vi "GOOP_AddCtrlToVIIfNeeded.vi"(11 "Ctrl VI in":refnum<vi>) -> (2 "error out":errorcluster, 3 "VI out":refnum<vi>, 5 "CtrlOut":refnum<vi>)   [LabVIEW 2020]
uses:
  <vilib>/Utility/miscctls.llb/LVPointTypeDef.ctl
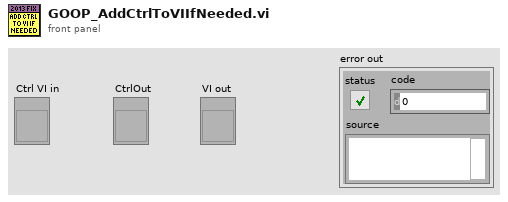
[diagram p1: front panel]
types:
  T1 = typedef "LVPointTypeDef.ctl" = cluster{"Horizontal":i16, "Vertical":i16}
  T2 = enum32{"invalid VI type", "Standard VI", "Control VI", "Global VI", "Polymorphic VI", "Configuration VI", "SubSystem", "Facade VI", "Method VI", "Statechart Diagram VI"}
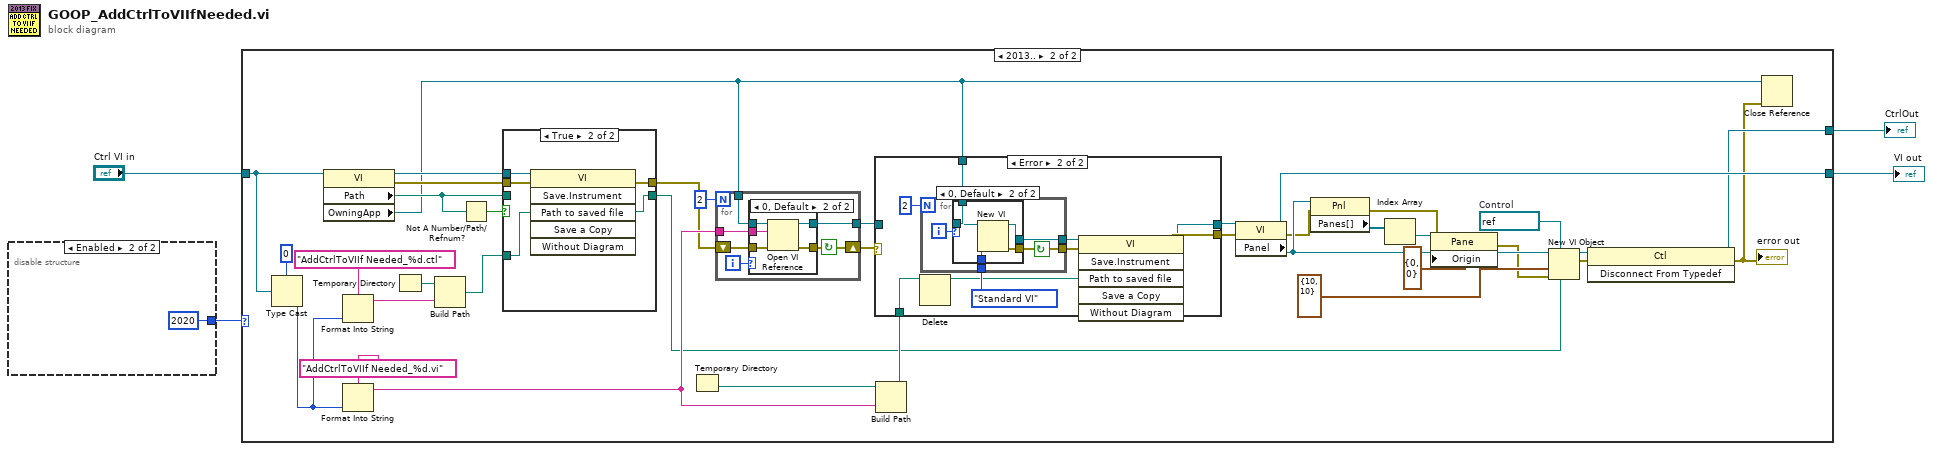
[diagram p0: block diagram]
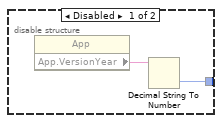
[diagram p2: hidden frame]
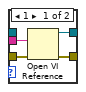
[diagram p4: hidden frame]
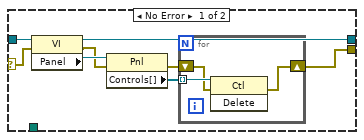
[diagram p6: hidden frame]
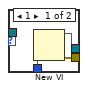
[diagram p7: hidden frame]
diagram:
  n1 = disable-structure shown="Enabled" {
    disable-tunnel: [w5 2020] -> w4
    frame Disabled {
      n2 = property class="App"() -> ("App.VersionYear"=w6:string)  [unwired: 2 in, 2 out]
      n3 = Decimal String To Number(string=w6) -> (number=w5:i32)  [unwired: 2 in, 1 out]
    }
    frame Enabled {
    }
  }
  n4 = case shown="2013.." w4 {
    tunnel: "Ctrl VI in" -> [w8 w29]
    tunnel: [w8 w34] -> w2
    tunnel: [_ w23] -> w1
    frame Default {
    }
    frame 2013.. {
      w33 = refnum<vi> refnum  # Control
      n5 = Type Cast(type=u32 0, x=w29) -> (*(type *) &x=w22:u32)
      n6 = property class="VI"(reference=w29) -> (reference out=w13:refnum<vi>, error out=w16:errorcluster, "Path"=w17:path, "OwningApp"=w10:refnum<vi>)  [unwired: 1 in]
      n7 = Format Into String(format string="AddCtrlToVIIf Needed_%d.ctl", w22) -> (resulting string=w20:string)  [unwired: 2 in, 1 out]
      n8 = Format Into String(format string="AddCtrlToVIIf Needed_%d.vi", w22) -> (resulting string=w27:string)  [unwired: 2 in, 1 out]
      n9 = Temporary Directory() -> (w19:path)
      n10 = Build Path(base path=w19, name or relative path=w20) -> (appended path=w12:path)
      n11 = Not A Number/Path/Refnum?(number/path/refnum=w17) -> (NaN/Path/Refnum?=w18:bool)
      n12 = case shown="True" w18 {
        tunnel: w17 -> [w62 _]
        tunnel: w16 -> [w61 w66]
        tunnel: [w62 w63] -> w15
        tunnel: [w61 w64] -> w14
        tunnel: w13 -> [_ w65]
        tunnel: w12 -> [_ w63]
        frame False {
        }
        frame True {
          n13 = invoke class="VI" method="Save.Instrument"(reference=w65, error in=w66, "Path to saved file"=w63) -> (error out=w64:errorcluster)  [unwired: 3 in, 5 out]
        }
      }
      n14 = Temporary Directory() -> (w45:path)
      n15 = for {
        N: 2 -> [_]
        tunnel: [w51] -> w43
        tunnel: w27 -> [w50]
        tunnel: w10 -> [w48]
        shift-right: [w47] -> w44
        shift-left: w14 -> [w49]
        i -> [w46]
        stop <- w47 continue-if-true
        n16 = case shown="0, Default" w46 {
          tunnel: [w55 w60] -> w51
          tunnel: w50 -> [w54 w59]
          tunnel: w49 -> [w53 w58]
          tunnel: w48 -> [_ w57]
          tunnel: [w52 w56] -> w47
          frame 1 {
            n17 = Open VI Reference(vi path=w54, error in (no error)=w53) -> (vi reference=w55:refnum<vi>, error out=w52:errorcluster)  [unwired: 4 in]
          }
          frame 0, Default {
            n18 = Open VI Reference(application reference (local)=w57, vi path=w59, error in (no error)=w58) -> (vi reference=w60:refnum<vi>, error out=w56:errorcluster)  [unwired: 3 in]
          }
        }
      }
      n19 = Build Path(base path=w45, name or relative path=w27) -> (appended path=w42:path)
      n20 = case shown="Error" w44 {
        selector: w44 -> [w69 _]
        tunnel: w43 -> [w74 _]
        tunnel: w42 -> [_ w79]
        tunnel: [w68 w82] -> w41
        tunnel: [w67 w84] -> w32
        tunnel: w10 -> [_ w80]
        frame No Error {
          n21 = property class="VI"(reference=w74, error in=w69) -> (reference out=w68:refnum<vi>, error out=w70:errorcluster, "Panel"=w73:refnum<vi>)
          n22 = property class="Pnl"(reference=w73, error in=w70) -> (error out=w71:errorcluster, "Controls[]"=w72:refnum<vi>[])  [unwired: 1 out]
          n23 = for {
            tunnel: w72 -> [w77] mode=indexing
            shift-right: [w75] -> w67
            shift-left: w71 -> [w76]
            n24 = invoke class="Ctl" method="Delete"(reference=w77, error in=w76) -> (error out=w75:errorcluster)  [unwired: 1 in, 2 out]
          }
        }
        frame Error {
          n25 = Delete(path (use dialog)=w79) -> (deleted path=w81:path)  [unwired: 4 in, 2 out]
          n26 = for {
            N: 2 -> [_]
            tunnel: [w87] -> w86
            tunnel: T2."Standard VI" ("vi type (standard vi)") -> [w91]
            tunnel: [w90] -> w83
            tunnel: w80 -> [w89]
            i -> [w88]
            stop <- w87 continue-if-true
            n27 = case shown="0, Default" w88 {
              tunnel: [w94 w98] -> w87
              tunnel: w91 -> [w93 w97]
              tunnel: [w92 w96] -> w90
              tunnel: w89 -> [_ w95]
              frame 1 {
                n28 = New VI(9:w93) -> (0:w94:errorcluster, 3:w92:refnum<vi>)  [unwired: 6 in]
              }
              frame 0, Default {
                n29 = New VI(9:w97, 11:w95) -> (0:w98:errorcluster, 3:w96:refnum<vi>)  [unwired: 5 in]
              }
            }
          }
          n30 = invoke class="VI" method="Save.Instrument"(reference=w83, error in=w86, "Path to saved file"=w81) -> (reference out=w82:refnum<vi>, error out=w84:errorcluster)  [unwired: 3 in, 4 out]
        }
      }
      n31 = property class="VI"(reference=w41, error in=w32) -> (reference out=w34:refnum<vi>, error out=w31:errorcluster, "Panel"=w39:refnum<vi>)
      n32 = property class="Pnl"(reference=w39, error in=w31) -> (error out=w30:errorcluster, "Panes[]"=w38:refnum<vi>[])  [unwired: 1 out]
      n33 = Index Array(array=w38) -> (element=w37:refnum<vi>)  [unwired: 1 in]
      n34 = property class="Pane"(reference=w37, error in=w30, "Origin"=T1 {"Horizontal"=0, "Vertical"=0}) -> (error out=w35:errorcluster)  [unwired: 1 out]
      n35 = New VI Object(vi object class=w33, owner refnum=w39, position/next to=T1 {"Horizontal"=10, "Vertical"=10} ("location"), 6:w15, 8:w35) -> (object refnum=w25:refnum<vi>, 0:w24:errorcluster)  [unwired: 3 in]
      n36 = invoke class="Ctl" method="Disconnect From Typedef"(reference=w25, error in=w24) -> (reference out=w23:refnum<vi>, error out=w11:errorcluster)  [unwired: 1 in, 1 out]
      "error out" <- w11
      n37 = Close Reference(reference=w10, error in (no error)=w11) -> ()  [unwired: 1 out]
    }
  }
  "VI out" <- w2
  "CtrlOut" <- w1
